vi "RPC Method ThermalChamberController SubscribeRampRateUpdated.vi"(8 "error in (no error)":errorcluster, 11 "gRPC service in":refnum<class "ThermalChamberController.lvclass">) -> (0 "error out":errorcluster, 3 "gRPC service out":refnum<class "ThermalChamberController.lvclass">)   [LabVIEW 2020, in "thermal-chamber-controller_server.lvlib" / "ThermalChamberController.lvclass"]
uses:
  ThermalChamberController.lvclass
  ThermalChamberController.lvclass/ThermalChamberController.ctl
  Program Files (x86)/National Instruments/LabVIEW 2020/examples/DQMH Consortium/DQMH Fundamentals - Thermal Chamber/Libraries/Thermal Chamber Controller_DQMH/Thermal Chamber Controller_DQMH.lvlib
  <vilib>/gRPC/LabVIEW gRPC Library/Shared/grpcId.ctl
  <vilib>/gRPC/LabVIEW gRPC Library/grpc-lvsupport-release.lvlib
  support/Stream Data--cluster.ctl
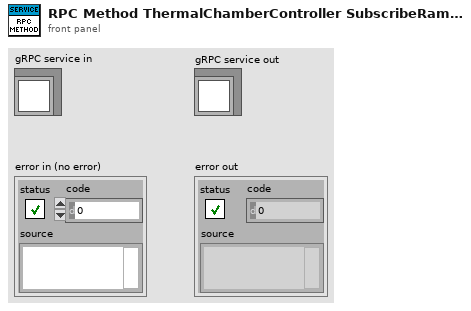
[diagram p1: front panel]
types:
  T1 = typedef "Stream Data--cluster.ctl" = cluster{"gRPCid":T2, "Active":bool, "timeout":i32}
  T2 = typedef "grpc-lvsupport-release.lvlib/grpcId.ctl" = u64
  T3 = typedef "thermal-chamber-controller_server.lvlib/ThermalChamberController.lvclass/Server Internal UEs.ctl" = cluster{"ThermalChamberController StartModule Internal UE":refnum<user-event>, "ThermalChamberController ShowModulePanel Internal UE":refnum<user-event>, "ThermalChamberController HideModulePanel Internal UE":refnum<user-event>, "ThermalChamberController StopModule Internal UE":refnum<user-event>, "ThermalChamberController UpdateSetPoint Internal UE":refnum<user-event>, "ThermalChamberController UpdateRampRate Internal UE":refnum<user-event>, "ThermalChamberController UpdateHeaterState Internal UE":refnum<user-event>, "ThermalChamberController SubscribeChamberStatusUpdated Internal UE":refnum<user-event>, "ThermalChamberController SubscribeSetPointUpdated Internal UE":refnum<user-event>, "ThermalChamberController SubscribeRampRateUpdated Internal UE":refnum<user-event>, "ThermalChamberController SubscribeHeaterStateUpdated Internal UE":refnum<user-event>}
  T4 = typedef "thermal-chamber-controller_server.lvlib/ThermalChamberController.lvclass/Server gRPC UEs.ctl" = cluster{"ThermalChamberController StartModule gRPC UE":refnum<user-event>, "ThermalChamberController ShowModulePanel gRPC UE":refnum<user-event>, "ThermalChamberController HideModulePanel gRPC UE":refnum<user-event>, "ThermalChamberController StopModule gRPC UE":refnum<user-event>, "ThermalChamberController UpdateSetPoint gRPC UE":refnum<user-event>, "ThermalChamberController UpdateRampRate gRPC UE":refnum<user-event>, "ThermalChamberController UpdateHeaterState gRPC UE":refnum<user-event>, "ThermalChamberController SubscribeChamberStatusUpdated gRPC UE":refnum<user-event>, "ThermalChamberController SubscribeSetPointUpdated gRPC UE":refnum<user-event>, "ThermalChamberController SubscribeRampRateUpdated gRPC UE":refnum<user-event>, "ThermalChamberController SubscribeHeaterStateUpdated gRPC UE":refnum<user-event>}
  T5 = typedef "Thermal Chamber Controller_DQMH.lvlib/Broadcast Events--cluster.ctl" = cluster{"Module Did Init":refnum<user-event>, "Status Updated":refnum<user-event>, "Error Reported":refnum<user-event>, "Module Did Stop":refnum<user-event>, "Update Module Execution Status":refnum<user-event>, "Chamber Status Updated":refnum<user-event>, "Set Point Updated":refnum<user-event>, "Ramp Rate Updated":refnum<user-event>, "Heater State Updated":refnum<user-event>}
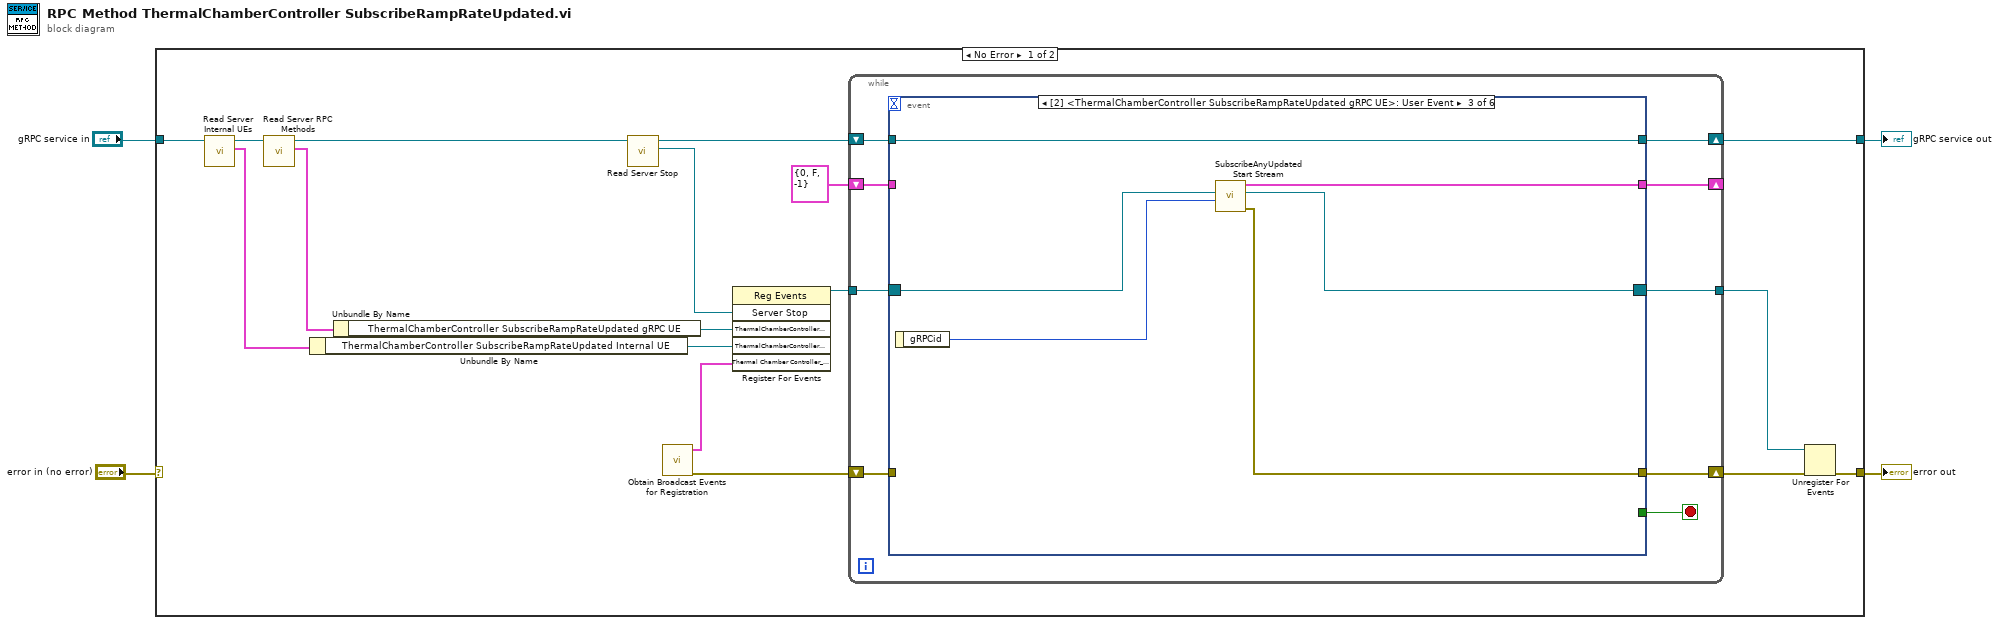
[diagram p0: block diagram]
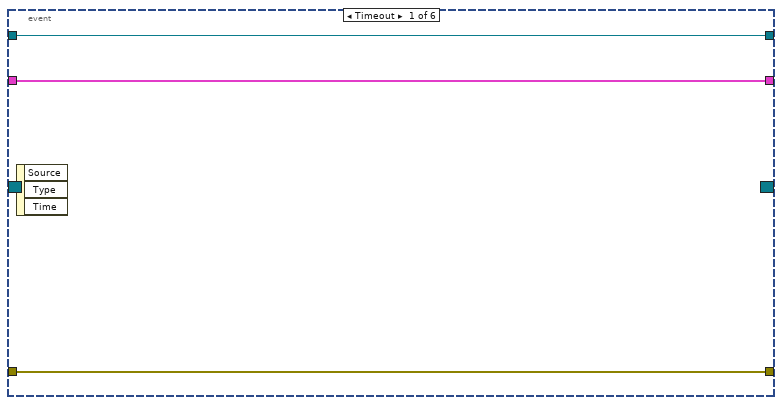
[diagram p2: hidden frame]
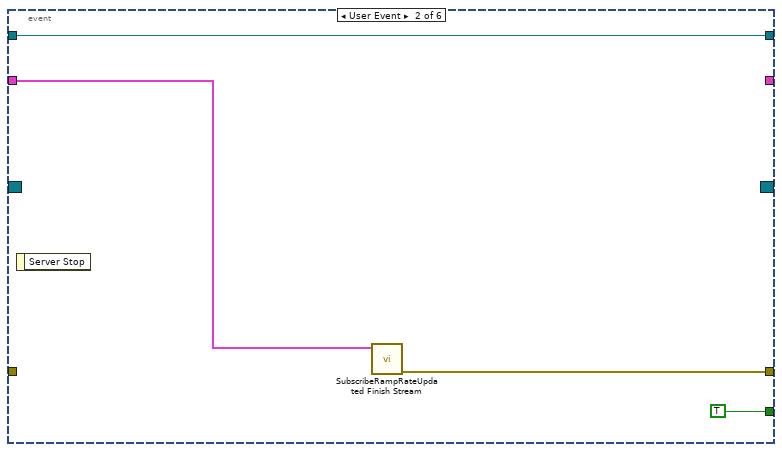
[diagram p3: hidden frame]
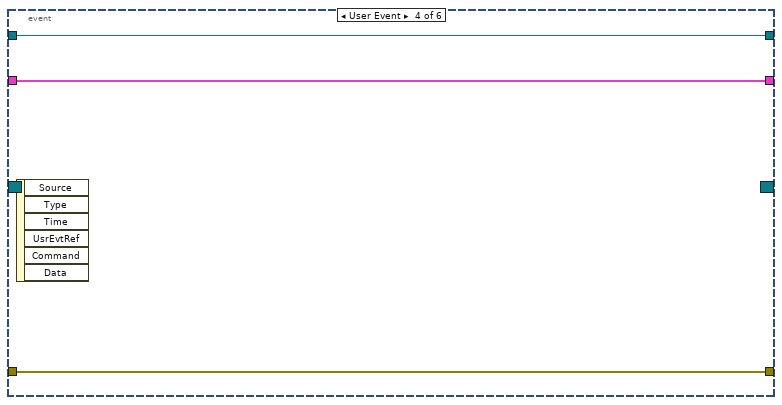
[diagram p4: hidden frame]
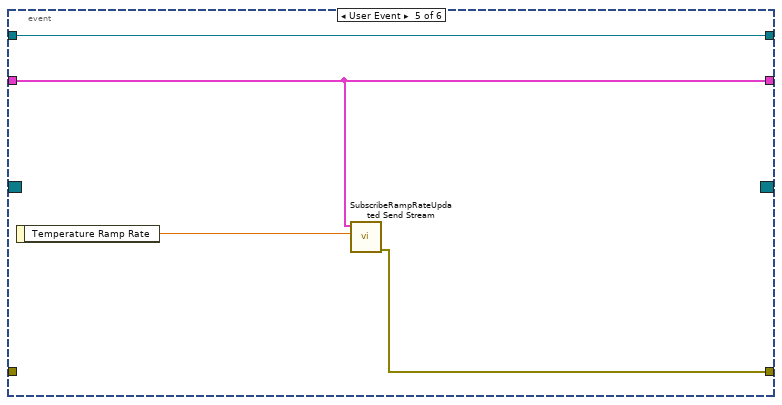
[diagram p5: hidden frame]
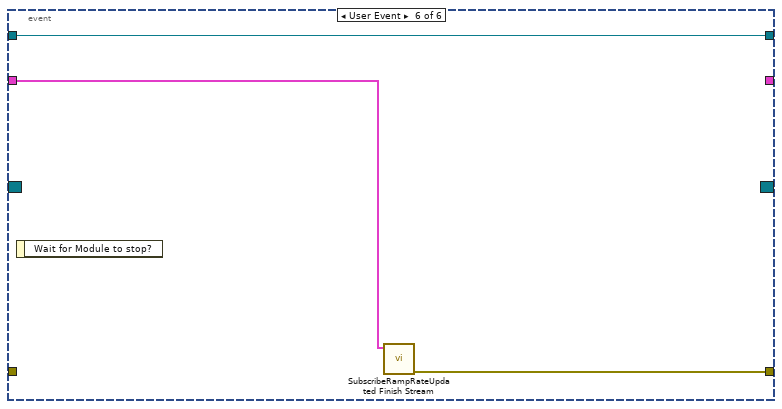
[diagram p6: hidden frame]
diagram:
  n1 = case shown="No Error" "error in (no error)" {
    selector: "error in (no error)" -> [_ w55]
    tunnel: [w16 w55] -> w3
    tunnel: "gRPC service in" -> [w19 w54]
    tunnel: [w8 w54] -> w1
    frame No Error {
      n2 = call "Read Server Internal UEs.vi"("gRPC service in"=w19) -> ("Server Internal UEs"=w12:T3, "gRPC service out"=w18:refnum<class "ThermalChamberController.lvclass">)  [unwired: 8 in, 1 out]
      n3 = call "Read Server RPC Methods.vi"("gRPC service in"=w18) -> ("Server RPC Methods"=w14:T4, "gRPC service out"=w9:refnum<class "ThermalChamberController.lvclass">)  [unwired: 8 in, 1 out]
      n4 = Unbundle By Name ("Unbundle Internal UE")(w12) -> ("ThermalChamberController SubscribeRampRateUpdated Internal UE"=w11:refnum<user-event>)
      n5 = Unbundle By Name ("Unbundle gRPC UE")(w14) -> ("ThermalChamberController SubscribeRampRateUpdated gRPC UE"=w13:refnum<user-event>)
      n6 = call-dynamic "Read Server Stop.vi"("gRPC service in"=w9) -> ("Server Stop"=w21:refnum<user-event>, "gRPC service out"=w10:refnum<class "ThermalChamberController.lvclass">)  [unwired: 8 in, 1 out]
      n7 = call "Obtain Broadcast Events for Registration.vi"() -> ("error out"=w7:errorcluster, "Thermal Chamber Controller_DQMH Broadcast Events"=w6:T5)  [unwired: 9 in, 1 out]
      n8 = register-events(w21, w13, w11, w6) -> (reference out=w20:refnum<event-registration>)  [unwired: 2 in, 1 out]
      n9 = while {
        tunnel: w20 -> [w30]
        tunnel: [w26] -> w15
        shift-right: [w27] -> w17
        shift-left: w7 -> [w28]
        shift-right: [w24] -> w8
        shift-left: w10 -> [w25]
        shift-right: [w22] -> _
        shift-left: T1 {"gRPCid"=0, "Active"=FALSE, "timeout"=-1} ("Stream Data") -> [w23]
        stop <- w29 stop-if-true
        n10 = event "RPC Method Event Structure" shown="[2] <ThermalChamberController SubscribeRampRateUpdated gRPC UE>: User Event" {
          selector: w30 -> [_ _ w41 _ _ _]
          dyn-events: [_ _ w40 _ _ _] -> w26
          timeout: _ -> [_ _ _ _ _ _]
          tunnel: [_ TRUE _ _ _ _] -> w29
          tunnel: w28 -> [w33 _ _ w46 _ _]
          tunnel: [w33 w34 w38 w46 w47 w51] -> w27
          tunnel: w25 -> [w32 w36 w43 w45 w50 w53]
          tunnel: [w32 w36 w43 w45 w50 w53] -> w24
          tunnel: w23 -> [w31 w35 _ w44 w49 w52]
          tunnel: [w31 _ w42 w44 w49 _] -> w22
          event Timeout {
            n11 = event-data() -> ()  [unwired: 1 in, 3 out]
          }
          event User Event {
            n12 = event-data() -> ()  [unwired: 1 in, 1 out]
            n13 = call "SubscribeRampRateUpdated Finish Stream.vi"("Stream Data in"=w35) -> ("error out"=w34:errorcluster)  [unwired: 10 in]
          }
          event User Event {
            n14 = event-data() -> ("gRPCid"=w39:T2)  [unwired: 1 in]
            n15 = call "SubscribeAnyUpdated Start Stream.vi"("gRPCid"=w39, "Event Registration Refnum in"=w41) -> ("error out"=w38:errorcluster, "Event Registration Refnum out"=w40:refnum<event-registration>, "Stream Data out"=w42:T1)  [unwired: 7 in]
          }
          event User Event {
            n16 = event-data() -> ()  [unwired: 1 in, 6 out]
          }
          event User Event {
            n17 = event-data() -> ("Temperature Ramp Rate"=w48:dbl)  [unwired: 1 in]
            n18 = call "SubscribeRampRateUpdated Send Stream.vi"("Temperature Ramp Rate"=w48, "Stream Data in"=w49) -> ("error out"=w47:errorcluster)  [unwired: 9 in]
          }
          event User Event {
            n19 = event-data() -> ()  [unwired: 1 in, 1 out]
            n20 = call "SubscribeRampRateUpdated Finish Stream.vi"("Stream Data in"=w52) -> ("error out"=w51:errorcluster)  [unwired: 10 in]
          }
        }
      }
      n21 = Unregister For Events(event registration refnum=w15, error in=w17) -> (error out=w16:errorcluster)
    }
    frame Error {
    }
  }
  "error out" <- w3
  "gRPC service out" <- w1
